vi "PhotonPoseEstimator_Update_All.vi"(9 "Has New Results":bool, 10 "PipelineResult":T1={"Targets"=[], "PhotonMultiTargetPNPResult"={"PhotonPNPResult"={"IsPresent"=FALSE, "bestReprojErr"=0.0, "altReprojErr"=0.0, "ambiguity"=0.0, "Best"={"TRANSLATION3D"={"X"=0.0, "Y"=0.0, "Z"=0.0}, "ROTATION3D"={"Q_quaternion"={"R"=1.0, "V"=[0.0, 0.0, 0.0]}}, "XF"=FALSE}, "Alt"={"TRANSLATION3D"={"X"=0.0, "Y"=0.0, "Z"=0.0}, "ROTATION3D"={"Q_quaternion"={"R"=1.0, "V"=[0.0, 0.0, 0.0]}}, "XF"=FALSE}}, "FiducialIDsUsed"=[]}, "PhotonPipelineMetadata"={"CaptureTimestampMicros"=0, "PublishTimestampMicros"=0, "SequenceID"=0, "TimeSinceLastPong"=0}} {"PhotonMultiTargetPNPResult"."PhotonPNPResult"."Alt"."TRANSLATION3D"."Z" format="%14.3f"; "PhotonMultiTargetPNPResult"."PhotonPNPResult"."Alt"."TRANSLATION3D"."Y" format="%14.3f"; "PhotonMultiTargetPNPResult"."PhotonPNPResult"."Alt"."TRANSLATION3D"."X" format="%14.3f"; "PhotonMultiTargetPNPResult"."PhotonPNPResult"."Best"."TRANSLATION3D"."Z" format="%14.3f"; "PhotonMultiTargetPNPResult"."PhotonPNPResult"."Best"."TRANSLATION3D"."Y" format="%14.3f"; "PhotonMultiTargetPNPResult"."PhotonPNPResult"."Best"."TRANSLATION3D"."X" format="%14.3f"; "Targets"."AltCameraToTarget"."TRANSLATION3D"."Z" format="%14.3f"; "Targets"."AltCameraToTarget"."TRANSLATION3D"."Y" format="%14.3f"; "Targets"."AltCameraToTarget"."TRANSLATION3D"."X" format="%14.3f"; "Targets"."BestCameraToTarget"."TRANSLATION3D"."Z" format="%14.3f"; "Targets"."BestCameraToTarget"."TRANSLATION3D"."Y" format="%14.3f"; "Targets"."BestCameraToTarget"."TRANSLATION3D"."X" format="%14.3f"}, 11 "PhotonPoseEstimator":T14={"LastPose"={"Translation3d"={"X"=0.0, "Y"=0.0, "Z"=0.0}, "Rotation3d"={"Q_quaternion"={"R"=1.0, "V"=[0.0, 0.0, 0.0]}}}, "ReferencePose"={"Translation3d"={"X"=0.0, "Y"=0.0, "Z"=0.0}, "Rotation3d"={"Q_quaternion"={"R"=1.0, "V"=[0.0, 0.0, 0.0]}}}, "FieldTags"={"AprilTagMap"={}, "FieldLength"=0.0, "FieldWidth"=0.0, "OriginPosition "=enum."kBlueAllianceWallRightSide,", "OriginPose3d"={"Translation3d"={"X"=0.0, "Y"=0.0, "Z"=0.0}, "Rotation3d"={"Q_quaternion"={"R"=1.0, "V"=[0.0, 0.0, 0.0]}}}}, "PrimaryStratety"=enum."LOWEST_AMBIGUITY", "Camera"="", "RobotToCamera"={"TRANSLATION3D"={"X"=0.0, "Y"=0.0, "Z"=0.0}, "ROTATION3D"={"Q_quaternion"={"R"=1.0, "V"=[0.0, 0.0, 0.0]}}, "XF"=FALSE}, "ReportedErrors"=[], "HighestAmbiguity"=10.0, "MultiTagFallbackStrategy"=enum."LOWEST_AMBIGUITY", "PoseCacheTimeoutSec"=-1.0, "PhotonTargetModel"={"Vertices"=[], "IsPlaner"=FALSE, "IsSpherical"=FALSE}, "BaseNTName"="/photonvision"} {"PhotonTargetModel"."Vertices"."Z" format="%14.3f"; "PhotonTargetModel"."Vertices"."Y" format="%14.3f"; "PhotonTargetModel"."Vertices"."X" format="%14.3f"; "RobotToCamera"."TRANSLATION3D"."Z" format="%14.3f"; "RobotToCamera"."TRANSLATION3D"."Y" format="%14.3f"; "RobotToCamera"."TRANSLATION3D"."X" format="%14.3f"; "FieldTags"."OriginPose3d"."Translation3d"."Z" format="%14.3f"; "FieldTags"."OriginPose3d"."Translation3d"."Y" format="%14.3f"; "FieldTags"."OriginPose3d"."Translation3d"."X" format="%14.3f"; "ReferencePose"."Translation3d"."Z" format="%14.3f"; "ReferencePose"."Translation3d"."Y" format="%14.3f"; "ReferencePose"."Translation3d"."X" format="%14.3f"; "LastPose"."Translation3d"."Z" format="%14.3f"; "LastPose"."Translation3d"."Y" format="%14.3f"; "LastPose"."Translation3d"."X" format="%14.3f"}) -> (1 "Pos Found":bool, 2 "PhotonEstimatedRobotPose":T11={"EstimatedPose"={"Translation3d"={"X"=0.0, "Y"=0.0, "Z"=0.0}, "Rotation3d"={"Q_quaternion"={"R"=1.0, "V"=[0.0, 0.0, 0.0]}}}, "TimeStamp_Seconds"=0.0, "targetsUsed"=[], "Strategy"=enum."LOWEST_AMBIGUITY"} {"targetsUsed"."AltCameraToTarget"."TRANSLATION3D"."Z" format="%14.3f"; "targetsUsed"."AltCameraToTarget"."TRANSLATION3D"."Y" format="%14.3f"; "targetsUsed"."AltCameraToTarget"."TRANSLATION3D"."X" format="%14.3f"; "targetsUsed"."BestCameraToTarget"."TRANSLATION3D"."Z" format="%14.3f"; "targetsUsed"."BestCameraToTarget"."TRANSLATION3D"."Y" format="%14.3f"; "targetsUsed"."BestCameraToTarget"."TRANSLATION3D"."X" format="%14.3f"; "EstimatedPose"."Translation3d"."Z" format="%14.3f"; "EstimatedPose"."Translation3d"."Y" format="%14.3f"; "EstimatedPose"."Translation3d"."X" format="%14.3f"}, 3 "out PhotonPoseEstimator":T14={"LastPose"={"Translation3d"={"X"=0.0, "Y"=0.0, "Z"=0.0}, "Rotation3d"={"Q_quaternion"={"R"=1.0, "V"=[0.0, 0.0, 0.0]}}}, "ReferencePose"={"Translation3d"={"X"=0.0, "Y"=0.0, "Z"=0.0}, "Rotation3d"={"Q_quaternion"={"R"=1.0, "V"=[0.0, 0.0, 0.0]}}}, "FieldTags"={"AprilTagMap"={}, "FieldLength"=0.0, "FieldWidth"=0.0, "OriginPosition "=enum."kBlueAllianceWallRightSide,", "OriginPose3d"={"Translation3d"={"X"=0.0, "Y"=0.0, "Z"=0.0}, "Rotation3d"={"Q_quaternion"={"R"=1.0, "V"=[0.0, 0.0, 0.0]}}}}, "PrimaryStratety"=enum."LOWEST_AMBIGUITY", "Camera"="", "RobotToCamera"={"TRANSLATION3D"={"X"=0.0, "Y"=0.0, "Z"=0.0}, "ROTATION3D"={"Q_quaternion"={"R"=1.0, "V"=[0.0, 0.0, 0.0]}}, "XF"=FALSE}, "ReportedErrors"=[], "HighestAmbiguity"=10.0, "MultiTagFallbackStrategy"=enum."LOWEST_AMBIGUITY", "PoseCacheTimeoutSec"=-1.0, "PhotonTargetModel"={"Vertices"=[], "IsPlaner"=FALSE, "IsSpherical"=FALSE}, "BaseNTName"="/photonvision"} {"PhotonTargetModel"."Vertices"."Z" format="%14.3f"; "PhotonTargetModel"."Vertices"."Y" format="%14.3f"; "PhotonTargetModel"."Vertices"."X" format="%14.3f"; "RobotToCamera"."TRANSLATION3D"."Z" format="%14.3f"; "RobotToCamera"."TRANSLATION3D"."Y" format="%14.3f"; "RobotToCamera"."TRANSLATION3D"."X" format="%14.3f"; "FieldTags"."OriginPose3d"."Translation3d"."Z" format="%14.3f"; "FieldTags"."OriginPose3d"."Translation3d"."Y" format="%14.3f"; "FieldTags"."OriginPose3d"."Translation3d"."X" format="%14.3f"; "ReferencePose"."Translation3d"."Z" format="%14.3f"; "ReferencePose"."Translation3d"."Y" format="%14.3f"; "ReferencePose"."Translation3d"."X" format="%14.3f"; "LastPose"."Translation3d"."Z" format="%14.3f"; "LastPose"."Translation3d"."Y" format="%14.3f"; "LastPose"."Translation3d"."X" format="%14.3f"})   [LabVIEW 2019, in "PhotonVisionLib.lvlib"]
doc: "Provided data from polling a camera, updates the estimated position of the robot. Returns empty if:\n - New data has not been received since the last call to update.\n - No targets were found from the camera\n - There is no camera set\n\n** DEPRECATED 2026 ** Functions that use the strategy enum are being deprecated. Use the individual strategy EXECUTE or ESTIMATE functions instead.\n\nInputs:\n -- PhotonPoseEstimator -- data cluster -- Data guiding how the position determination is done.\n -- PipelineResults -- data cluster -- Data provided from PhotonCamera_GetLatestResults.\n -- HasResults -- boolean - TRUE if targets have been identified in the Pipeline results. This can be provided by PhotonCamera_GetLatestResults.\n -- cameraMatrix -- matrix -- Camera calibration data that can be used in the case of no assigned PhotonCamera.\n -- distCoeffs -- matrix -- Camera calibration data that can be used in the case of no assigned PhotonCamera\n\nOutputs:\n -- PhotonPoseEstimator -- data cluster -- Updated data cluster.\n -- PhotonEstimatedRobotPose -- data cluster -- Estimated robot position, timestamp, and targets used to create the estimte.\n -- PosFound -- boolean -- A position has been determined."
uses:
  PhotonVisionLib.lvlib
  TypeDef/PhotonPoseEstimatorType.ctl
  <vilib>/Rock Robotics/WPI/ThirdParty/JAS_Junk/TrajLib/TypeDef/POSE3D.ctl
  <vilib>/Rock Robotics/WPI/ThirdParty/JAS_Junk/TrajLib/TypeDef/TRANSLATION3D.ctl
  <vilib>/Rock Robotics/WPI/ThirdParty/JAS_Junk/TrajLib/TypeDef/ROTATION3D.ctl
  <vilib>/Rock Robotics/WPI/ThirdParty/JAS_Junk/TrajLib/TypeDef/QUATERNION.ctl
  <vilib>/Rock Robotics/WPI/ThirdParty/JAS_Junk/TrajLib/TypeDef/AprilTagFieldLayout.ctl
  <vilib>/Rock Robotics/WPI/ThirdParty/JAS_Junk/TrajLib/TypeDef/AprilTag.ctl
  <vilib>/Rock Robotics/WPI/ThirdParty/JAS_Junk/TrajLib/Enum/AprilTagFieldLayoutOrignPosition_ENUM.ctl
  Enum/PhotonPoseStrategy_ENUM.ctl
  <vilib>/Rock Robotics/WPI/ThirdParty/JAS_Junk/TrajLib/TypeDef/TRANSFORM3D.ctl
  TypeDef/PhotonTargetModel.ctl
  TypeDef/PhotonEstimatedRobotPoseType.ctl
  TypeDef/PhotonTrackedTargetType.ctl
  TypeDef/TargetCornerType.ctl
  TypeDef/PhotonPipelineResultType.ctl
  TypeDef/PhotonMultiTargetPNPResultType.ctl
  TypeDef/PhotonPNPResultType.ctl
  TypeDef/PhotonPipelineMetadataType.ctl
  <vilib>/Rock Robotics/WPI/ThirdParty/JAS_Junk/TrajLib/VI/Rotation3d_Create_AxisAngle.vi
  <vilib>/Rock Robotics/WPI/ThirdParty/JAS_Junk/TrajLib/VI/Pose3d_New.vi
  PhotonPipelineResult_HasTargets.vi
  PhotonPipelineResult_GetTargets.vi
  PhotonTrackedTarget_GetPoseAmbiguity.vi
  PhotonTrackedTarget_GetFiducialId.vi
  PhotonPoseEstimator_GetFieldTags.vi
  <vilib>/Rock Robotics/WPI/ThirdParty/JAS_Junk/TrajLib/VI/AprilTagFieldLayout_GetTagPose.vi
  <vilib>/Rock Robotics/WPI/ThirdParty/JAS_Junk/TrajLib/VI/Pose3d_TransformBy.vi
  PhotonTrackedTarget_GetBestCameraToTarget.vi
  <vilib>/Rock Robotics/WPI/ThirdParty/JAS_Junk/TrajLib/VI/Transform3d_Inverse.vi
  PhotonPoseEstimator_GetRobotToCameraTransform.vi
  PhotonPoseEstimator_GetHighestAmbiguity.vi
  PhotonEstimatedRobotPose_New.vi
  PhotonPoseEstimator_Strategy_closestToCameraHeight_calc.vi
  PhotonTrackedTarget_GetAltCameraToTarget.vi
  PhotonPoseEstimator_Strategy_closestToReferencePose_calc.vi
  PhotonPoseEstimator_Strategy_averageBestTargets_calc.vi
  <vilib>/Rock Robotics/WPI/ThirdParty/JAS_Junk/TrajLib/VI/Rotation3d_Plus.vi
  <vilib>/Rock Robotics/WPI/ThirdParty/JAS_Junk/TrajLib/VI/Translation3d_Plus.vi
  <vilib>/Rock Robotics/WPI/ThirdParty/JAS_Junk/TrajLib/VI/Translation3d_Times.vi
  <vilib>/Rock Robotics/WPI/ThirdParty/JAS_Junk/TrajLib/VI/Rotation3d_Times.vi
  <vilib>/Rock Robotics/WPI/ThirdParty/JAS_Junk/TrajLib/VI/Rotation3d_Create_Default.vi
  <vilib>/Rock Robotics/WPI/ThirdParty/JAS_Junk/TrajLib/VI/Translation3d_Create_Default.vi
  <vilib>/Rock Robotics/WPI/ThirdParty/JAS_Junk/TrajLib/VI/Pose3d_New_Trans3dRot3d.vi
  <vilib>/Rock Robotics/WPI/ThirdParty/JAS_Junk/TrajLib/VI/Pose3d_New_Default.vi
  <vilib>/Rock Robotics/WPI/ThirdParty/JAS_Junk/TrajLib/VI/Pose3d_Plus.vi
  <vilib>/Rock Robotics/WPI/ThirdParty/JAS_Junk/TrajLib/VI/Pose3d_RelativeTo.vi
  <vilib>/Rock Robotics/WPI/ThirdParty/JAS_Junk/TrajLib/VI/AprilTagFieldLayout_GetOriginPosition.vi
  PhotonPipelineResult_GetMultiTagResult.vi
  PhotonPipelineResult_GetBestTarget.vi
  PhotonTrackedTarget_GetPitch.vi
  PhotonTrackedTarget_GetYaw.vi
  <vilib>/Rock Robotics/WPI/ThirdParty/JAS_Junk/TrajLib/VI/Rotation3d_Create_RollPitchYaw.vi
  <vilib>/Rock Robotics/WPI/ThirdParty/JAS_Junk/TrajLib/Units_DegreesToRadians.vi
  <vilib>/Rock Robotics/WPI/ThirdParty/JAS_Junk/TrajLib/VI/Transform3d_GetTranslation3d.vi
  <vilib>/Rock Robotics/WPI/ThirdParty/JAS_Junk/TrajLib/VI/Translation3d_GetNorm.vi
  <vilib>/Rock Robotics/WPI/ThirdParty/JAS_Junk/TrajLib/VI/Translation3d_Create_DistAng.vi
  <vilib>/Rock Robotics/WPI/ThirdParty/JAS_Junk/TrajLib/VI/Translation3d_RotateBy.vi
  <vilib>/Rock Robotics/WPI/ThirdParty/JAS_Junk/TrajLib/VI/Translation3d_ToTranslation2d.vi
  <vilib>/Rock Robotics/WPI/ThirdParty/JAS_Junk/TrajLib/Translation2d_RotateBy.vi
  <vilib>/Rock Robotics/WPI/ThirdParty/JAS_Junk/TrajLib/VI/Transform3d_GetRotation3d.vi
  <vilib>/Rock Robotics/WPI/ThirdParty/JAS_Junk/TrajLib/VI/Pose3d_ToPose2d.vi
  <vilib>/Rock Robotics/WPI/ThirdParty/JAS_Junk/TrajLib/Pose2d_getTranslation.vi
  <vilib>/Rock Robotics/WPI/ThirdParty/JAS_Junk/TrajLib/Translation2d_Plus.vi
  <vilib>/Rock Robotics/WPI/ThirdParty/JAS_Junk/TrajLib/Translation2d_UnaryMinus.vi
  <vilib>/Rock Robotics/WPI/ThirdParty/JAS_Junk/TrajLib/Pose2d_New_TRRO.vi
  <vilib>/Rock Robotics/WPI/ThirdParty/JAS_Junk/TrajLib/VI/Pose3d_New_Pose2d.vi
  <vilib>/Rock Robotics/WPI/ThirdParty/JAS_Junk/TrajLib/VI/TimeInterpRotation2d_GetSample.vi
  PhotonPoseEstimator_GetHeadingBuffer.vi
  <vilib>/Rock Robotics/WPI/ThirdParty/JAS_Junk/TrajLib/VI/Quaternion_New.vi
  <vilib>/Rock Robotics/WPI/ThirdParty/JAS_Junk/TrajLib/VI/Vector_Norm.vi
  <vilib>/Rock Robotics/WPI/ThirdParty/JAS_Junk/TrajLib/VecBuilder_ArrayBy1Fill.vi
  <vilib>/Rock Robotics/WPI/ThirdParty/JAS_Junk/TrajLib/VI/Translation3d_Create.vi
  PhotonPipelineResult_GetTargetCount.vi
  <vilib>/Rock Robotics/WPI/ThirdParty/JAS_Junk/TrajLib/VI/AprilTag_GetAll.vi
  <vilib>/Rock Robotics/WPI/ThirdParty/JAS_Junk/TrajLib/VI/Pose3d_getTranslation3d.vi
  <vilib>/Rock Robotics/WPI/ThirdParty/JAS_Junk/TrajLib/VI/Pose3d_getRotation3d.vi
  <vilib>/Rock Robotics/WPI/ThirdParty/JAS_Junk/TrajLib/VI/Rotation3d_ToRotation2d.vi
  <vilib>/Rock Robotics/WPI/ThirdParty/JAS_Junk/TrajLib/Transform2d_Create_TransRot.vi
  <vilib>/Rock Robotics/WPI/ThirdParty/JAS_Junk/TrajLib/VI/Transform3d_Create_Trans3dRot3d.vi
  <vilib>/Rock Robotics/WPI/ThirdParty/JAS_Junk/TrajLib/VI/Rotation3d_UnaryMinus.vi
  <vilib>/Rock Robotics/WPI/ThirdParty/JAS_Junk/TrajLib/VI/Translation3d_UnaryMinus.vi
  <vilib>/Rock Robotics/WPI/ThirdParty/JAS_Junk/TrajLib/VI/Transform3d_GetXYZ.vi
  <vilib>/Rock Robotics/WPI/ThirdParty/JAS_Junk/TrajLib/VI/Pose3d_getXYZ.vi
  PhotonPoseEstimator_CalcDifference.vi
  <vilib>/Rock Robotics/WPI/ThirdParty/JAS_Junk/TrajLib/VI/Rotation3d_RotateBy.vi
  <vilib>/Rock Robotics/WPI/ThirdParty/JAS_Junk/TrajLib/VI/Translation3d_GetXYZ.vi
  <vilib>/Rock Robotics/WPI/ThirdParty/JAS_Junk/TrajLib/VI/Rotation3d_GetQuaterion.vi
  <vilib>/Rock Robotics/WPI/ThirdParty/JAS_Junk/TrajLib/VI/Quaternion_Get_Vect.vi
  <vilib>/Rock Robotics/WPI/ThirdParty/JAS_Junk/TrajLib/VI/Quaternion_Get_W.vi
  <vilib>/Rock Robotics/WPI/ThirdParty/JAS_Junk/TrajLib/VI/Quaternion_New_Default.vi
  <vilib>/Rock Robotics/WPI/ThirdParty/JAS_Junk/TrajLib/VI/Transform3d_Create_Pose3dPose3d.vi
  <vilib>/Rock Robotics/WPI/ThirdParty/JAS_Junk/TrajLib/Conv_Deg_Radians.vi
  <vilib>/Rock Robotics/WPI/ThirdParty/JAS_Junk/TrajLib/VI/Quaternion_Times.vi
  <vilib>/Rock Robotics/WPI/ThirdParty/JAS_Junk/TrajLib/VI/Quaternion_Inverse.vi
  <vilib>/Rock Robotics/WPI/ThirdParty/JAS_Junk/TrajLib/VI/Quaternion_Get_All.vi
  <vilib>/Rock Robotics/WPI/ThirdParty/JAS_Junk/TrajLib/Translation2d_Create.vi
  <vilib>/Rock Robotics/WPI/ThirdParty/JAS_Junk/TrajLib/Pose2d_getXYAngle.vi
  <vilib>/Rock Robotics/WPI/ThirdParty/JAS_Junk/TrajLib/Rotation2d_Interpolate.vi
  <vilib>/Rock Robotics/WPI/ThirdParty/JAS_Junk/TrajLib/MatBuilder_Create.vi
  <vilib>/Rock Robotics/WPI/ThirdParty/JAS_Junk/TrajLib/Rotation2d_CreateAngle.vi
  <vilib>/Rock Robotics/WPI/ThirdParty/JAS_Junk/TrajLib/VI/Rotation3d_GetXYZ.vi
  <vilib>/Rock Robotics/WPI/ThirdParty/JAS_Junk/TrajLib/VI/Rotation3d_Create_Quaternion.vi
  <vilib>/Rock Robotics/WPI/ThirdParty/JAS_Junk/TrajLib/VI/Translation3d_GetDistance.vi
  <vilib>/Rock Robotics/WPI/ThirdParty/JAS_Junk/TrajLib/VI/Translation3d_Minus.vi
  <vilib>/Rock Robotics/WPI/ThirdParty/JAS_Junk/TrajLib/VI/Rotation3d_Minus.vi
  <vilib>/Rock Robotics/WPI/ThirdParty/JAS_Junk/TrajLib/Rotation2d_Plus.vi
  <vilib>/Rock Robotics/WPI/ThirdParty/JAS_Junk/TrajLib/Rotation2d_Minus.vi
  <vilib>/Rock Robotics/WPI/ThirdParty/JAS_Junk/TrajLib/MathUtil_Clamp.vi
  <vilib>/Rock Robotics/WPI/ThirdParty/JAS_Junk/TrajLib/Rotation2d_Times.vi
  <vilib>/Rock Robotics/WPI/ThirdParty/JAS_Junk/TrajLib/VI/Quaternion_Normalize.vi
  <vilib>/Rock Robotics/WPI/ThirdParty/JAS_Junk/TrajLib/Rotation2d_RotateBy.vi
  <vilib>/Rock Robotics/WPI/ThirdParty/JAS_Junk/TrajLib/Rotation2d_UnaryMinus.vi
  <vilib>/Rock Robotics/WPI/ThirdParty/JAS_Junk/TrajLib/Rotation2d_CreateXY.vi
  <vilib>/Rock Robotics/WPI/ThirdParty/JAS_Junk/TrajLib/Util_CalcDist.vi
  PhotonVision_Globals.vi
  <vilib>/gmath/interp.llb/Search Ordered Table.vi
  <vilib>/Rock Robotics/WPI/ThirdParty/JAS_Junk/TrajLib/Trajectory_Library.lvlib
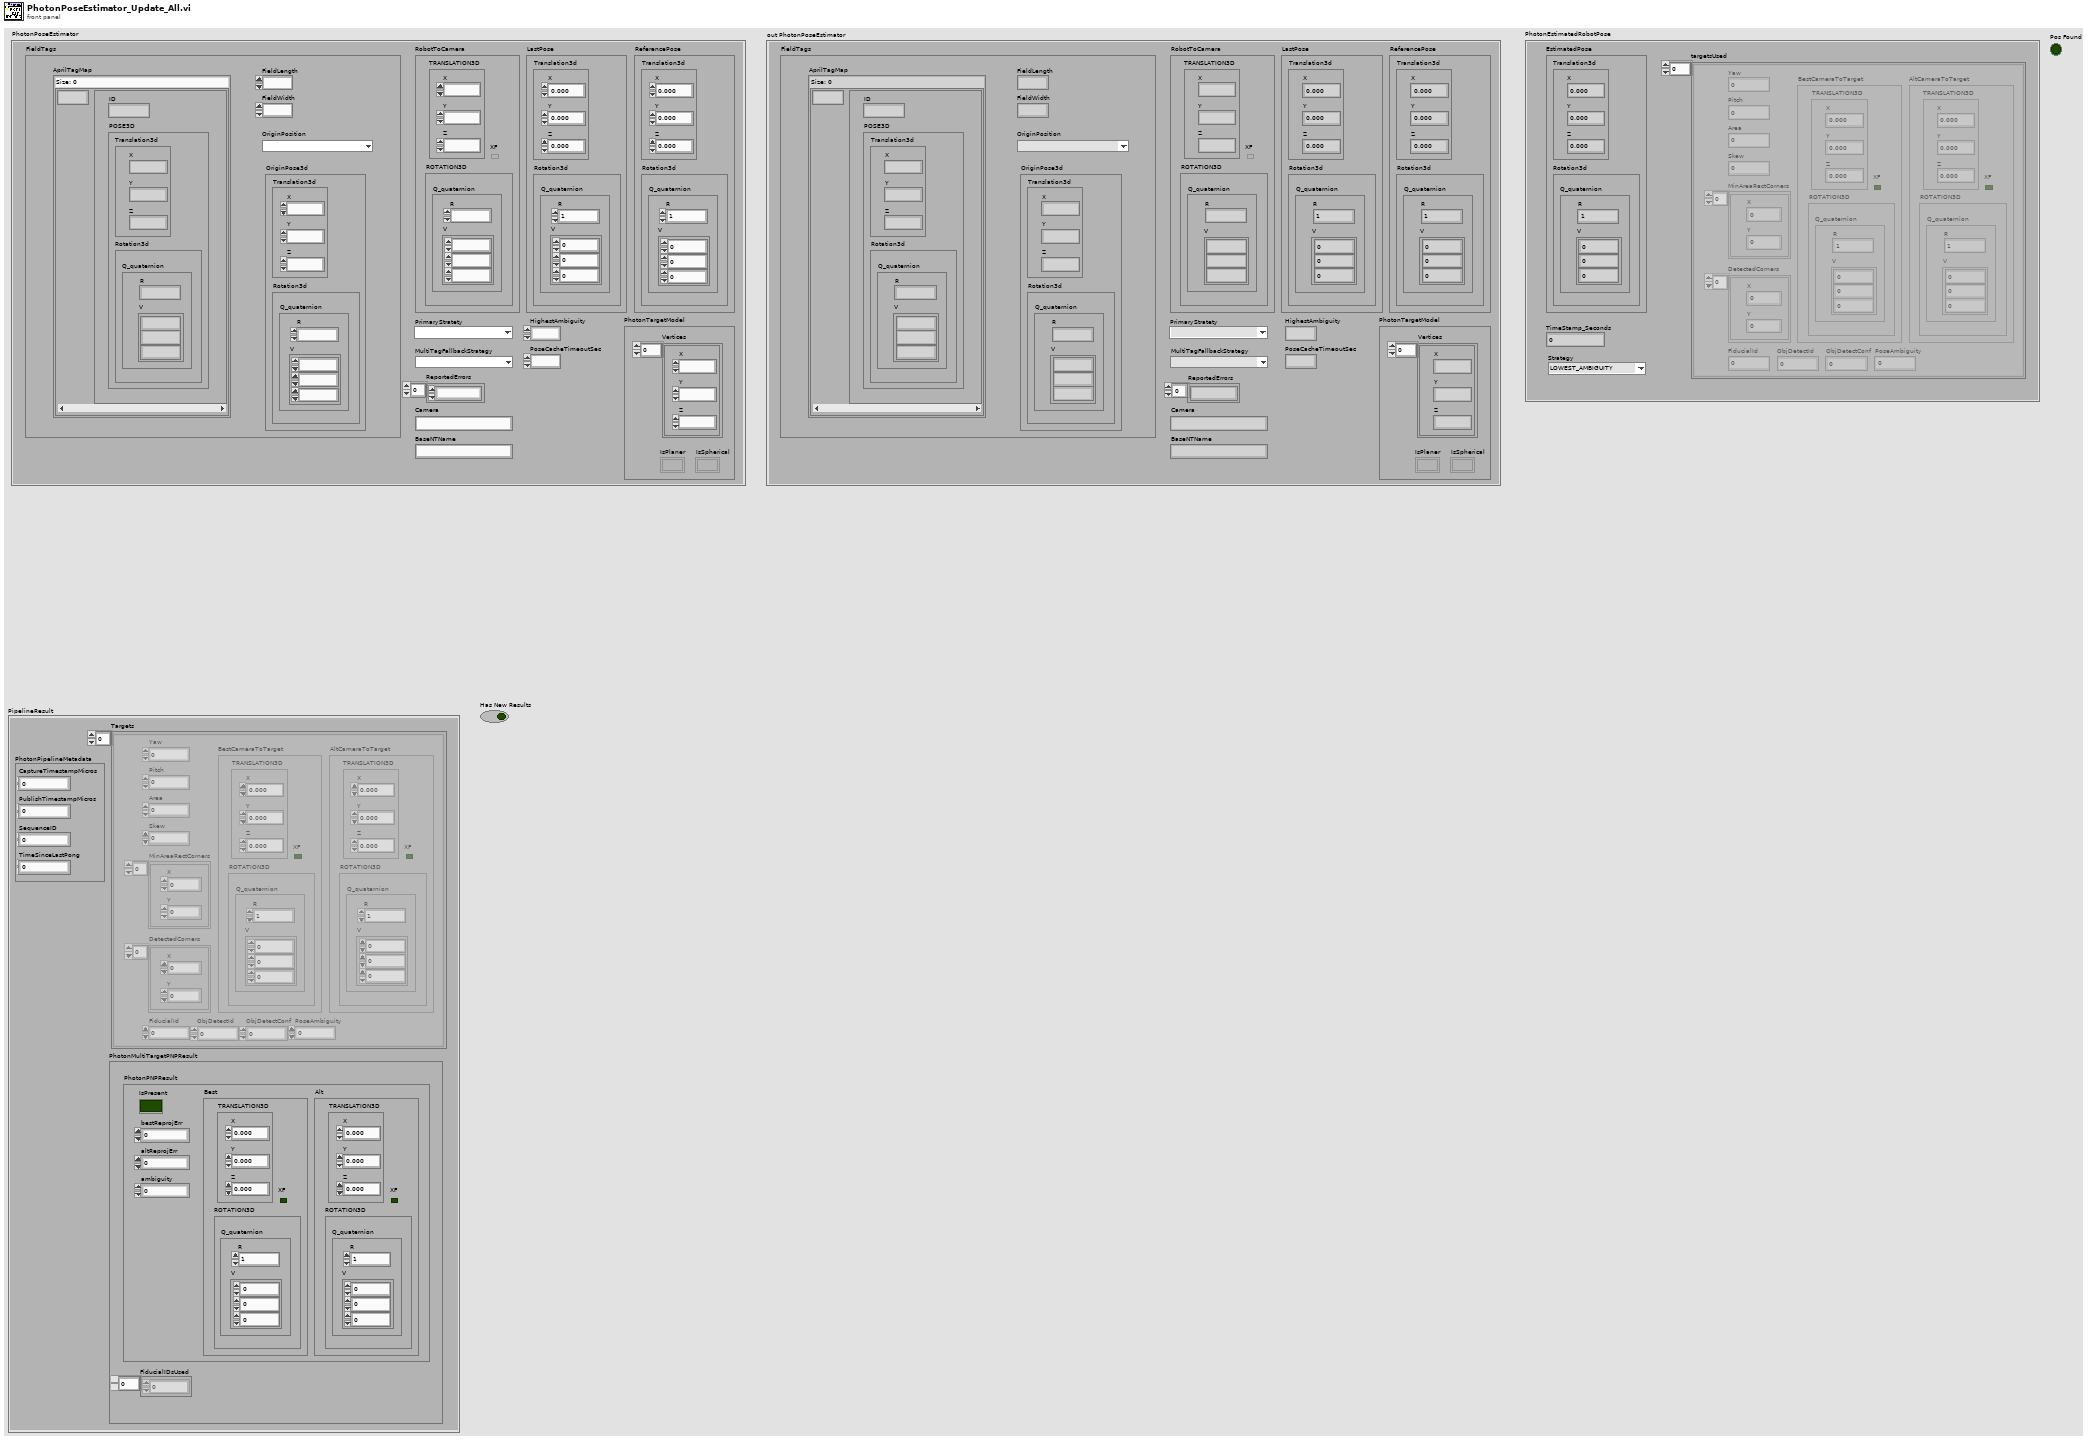
[diagram p1: front panel]
types:
  T1 = typedef "PhotonVisionLib.lvlib/PhotonPipelineResultType.ctl" = cluster{"Targets":T2[], "PhotonMultiTargetPNPResult":T8, "PhotonPipelineMetadata":T10}
  T2 = typedef "PhotonVisionLib.lvlib/PhotonTrackedTargetType.ctl" = cluster{"Yaw":dbl, "Pitch":dbl, "Area":dbl, "Skew":dbl, "MinAreaRectCorners":T3[], "BestCameraToTarget":T4, "FiducialId":i32, "AltCameraToTarget":T4, "PoseAmbiguity":dbl, "DetectedCorners":T3[], "ObjDetectId":i32, "ObjDetectConf":sgl}
  T3 = typedef "PhotonVisionLib.lvlib/TargetCornerType.ctl" = cluster{"X":dbl, "Y":dbl}
  T4 = typedef "Trajectory_Library.lvlib/TRANSFORM3D.ctl" = cluster{"TRANSLATION3D":T5, "ROTATION3D":T6, "XF":bool}
  T5 = typedef "Trajectory_Library.lvlib/TRANSLATION3D.ctl" = cluster{"X":dbl, "Y":dbl, "Z":dbl}
  T6 = typedef "Trajectory_Library.lvlib/ROTATION3D.ctl" = cluster{"Q_quaternion":T7}
  T7 = typedef "Trajectory_Library.lvlib/QUATERNION.ctl" = cluster{"R":dbl, "V":dbl[]}
  T8 = typedef "PhotonVisionLib.lvlib/PhotonMultiTargetPNPResultType.ctl" = cluster{"PhotonPNPResult":T9, "FiducialIDsUsed":i16[]}
  T9 = typedef "PhotonVisionLib.lvlib/PhotonPNPResultType.ctl" = cluster{"IsPresent":bool, "bestReprojErr":dbl, "altReprojErr":dbl, "ambiguity":dbl, "Best":T4, "Alt":T4}
  T10 = typedef "PhotonVisionLib.lvlib/PhotonPipelineMetadataType.ctl" = cluster{"CaptureTimestampMicros":i64, "PublishTimestampMicros":i64, "SequenceID":i64, "TimeSinceLastPong":i64}
  T11 = typedef "PhotonVisionLib.lvlib/PhotonEstimatedRobotPoseType.ctl" = cluster{"EstimatedPose":T12, "TimeStamp_Seconds":dbl, "targetsUsed":T2[], "Strategy":T13}
  T12 = typedef "Trajectory_Library.lvlib/POSE3D.ctl" = cluster{"Translation3d":T5, "Rotation3d":T6}
  T13 = typedef "PhotonVisionLib.lvlib/PhotonPoseStrategy_ENUM.ctl" = enum16{"LOWEST_AMBIGUITY", "CLOSEST_TO_CAMERA_HEIGHT", "CLOSEST_TO_REFERENCE_POSE", "CLOSEST_TO_LAST_POSE", "AVERAGE_BEST_TARGETS", "MULTI_TAG_PNP_ON_COPROCESSOR", "MULTI_TAG_PNP_ON_RIO", "PNP_DISTANCE_TRIG_SOLVE", "CONSTRAINED_SOLVEPNP"}
  T14 = typedef "PhotonVisionLib.lvlib/PhotonPoseEstimatorType.ctl" = cluster{"LastPose":T12, "ReferencePose":T12, "FieldTags":T15, "PrimaryStratety":T13, "Camera":string, "RobotToCamera":T4, "ReportedErrors":dbl[], "HighestAmbiguity":dbl, "MultiTagFallbackStrategy":T13, "PoseCacheTimeoutSec":dbl, "PhotonTargetModel":T18, "BaseNTName":string}
  T15 = typedef "Trajectory_Library.lvlib/AprilTagFieldLayout.ctl" = cluster{"AprilTagMap":map{i32, T16}, "FieldLength":dbl, "FieldWidth":dbl, "OriginPosition ":T17, "OriginPose3d":T12}
  T16 = typedef "Trajectory_Library.lvlib/AprilTag.ctl" = cluster{"ID":i32, "POSE3D":T12}
  T17 = typedef "Trajectory_Library.lvlib/AprilTagFieldLayoutOrignPosition_ENUM.ctl" = enum16{"kBlueAllianceWallRightSide,", "kRedAllianceWallRightSide,"}
  T18 = typedef "PhotonVisionLib.lvlib/PhotonTargetModel.ctl" = cluster{"Vertices":T5[], "IsPlaner":bool, "IsSpherical":bool}
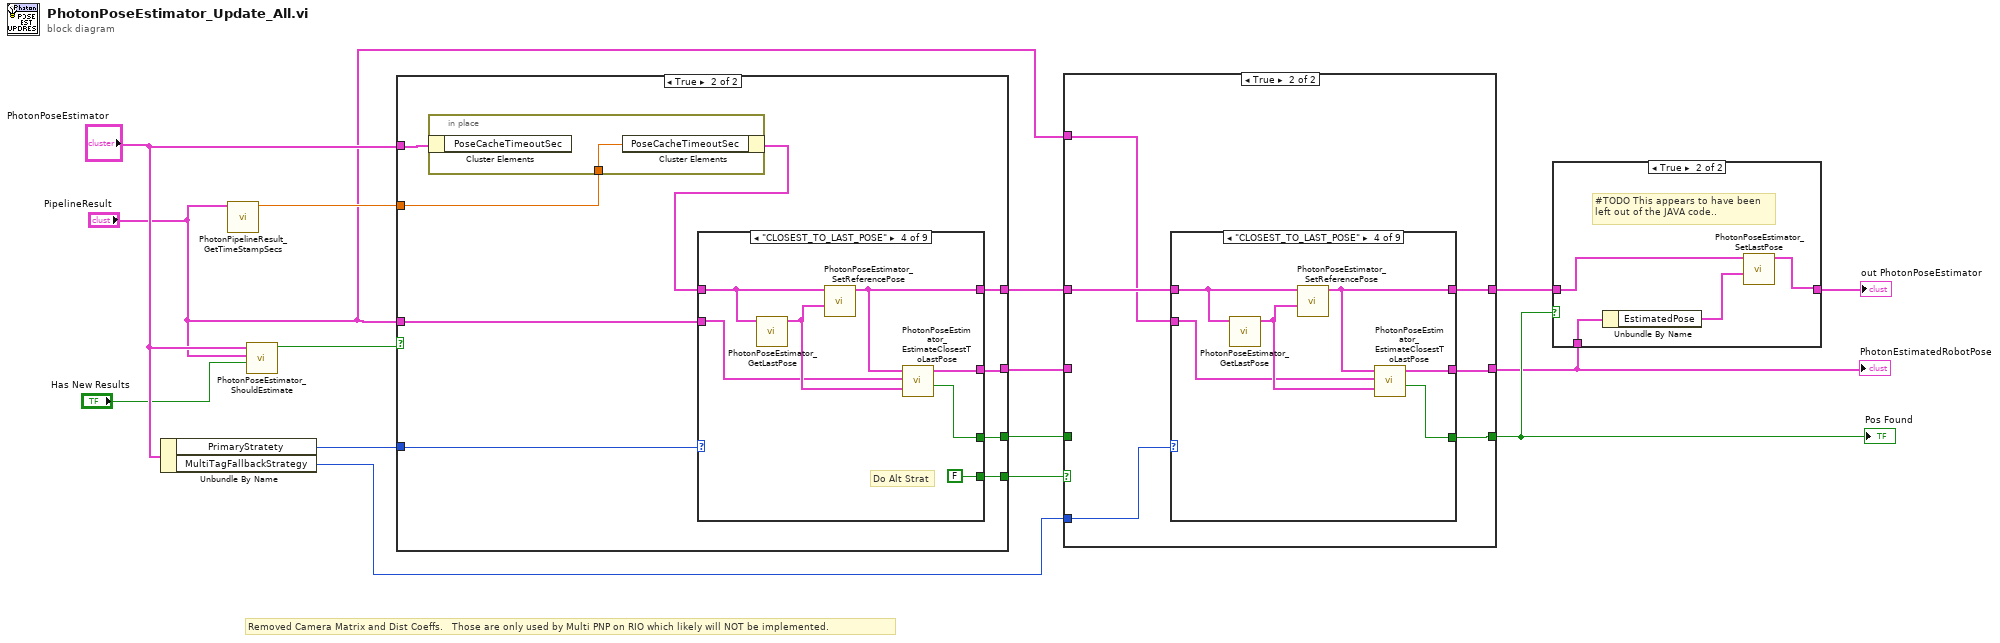
[diagram p0: block diagram]
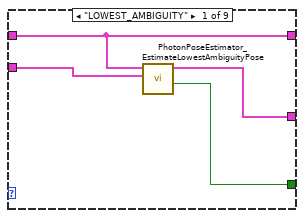
[diagram p3: hidden frame]
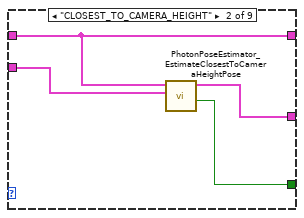
[diagram p4: hidden frame]
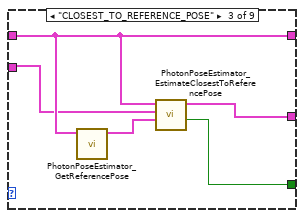
[diagram p5: hidden frame]
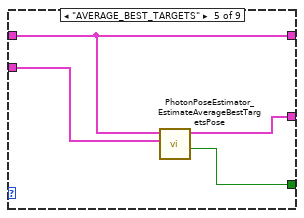
[diagram p6: hidden frame]
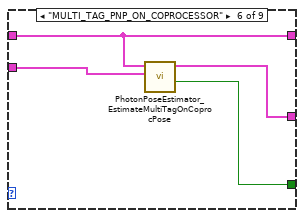
[diagram p7: hidden frame]
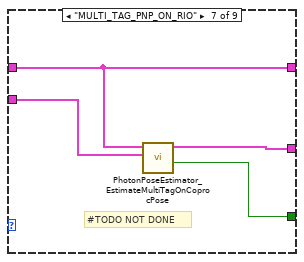
[diagram p8: hidden frame]
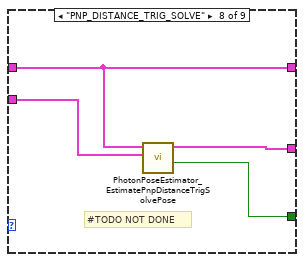
[diagram p9: hidden frame]
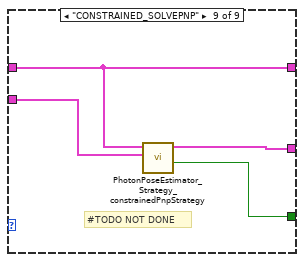
[diagram p10: hidden frame]
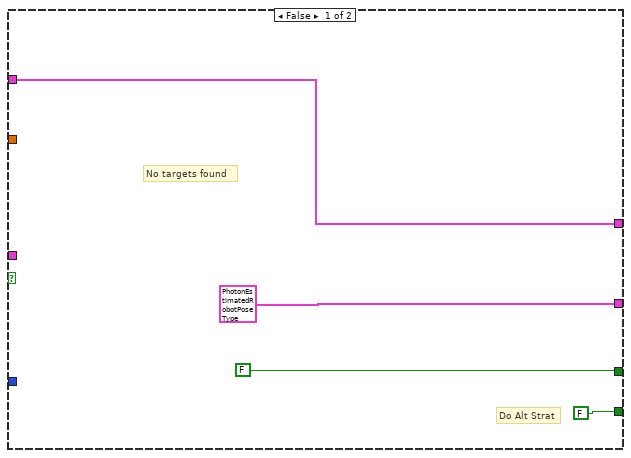
[diagram p11: hidden frame]
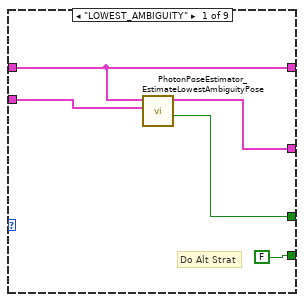
[diagram p12: hidden frame]
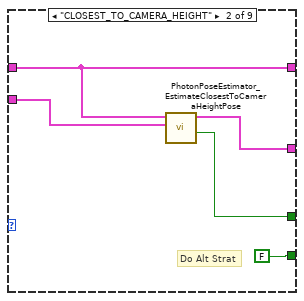
[diagram p13: hidden frame]
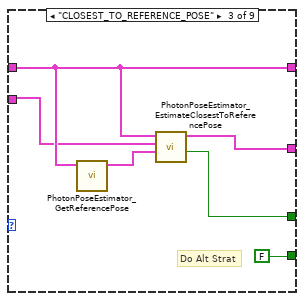
[diagram p14: hidden frame]
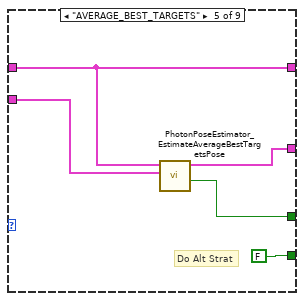
[diagram p15: hidden frame]
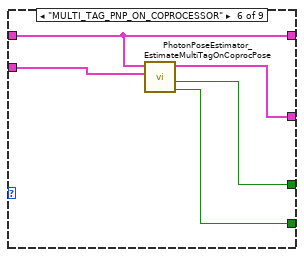
[diagram p16: hidden frame]
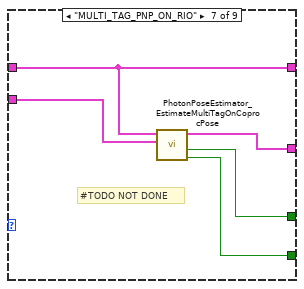
[diagram p17: hidden frame]
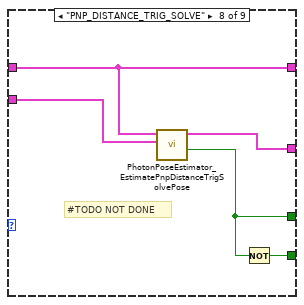
[diagram p18: hidden frame]
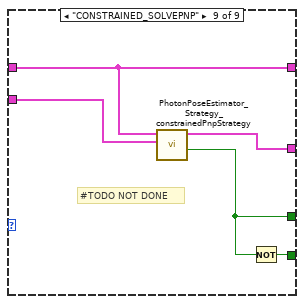
[diagram p19: hidden frame]
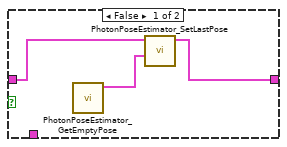
[diagram p20: hidden frame]
diagram:
  # "Removed Camera Matrix and Dist Coeffs.   Those are only used by Multi PNP on RIO which likely will NOT be implemented."
  n1 = Unbundle By Name("PhotonPoseEstimator") -> ("PrimaryStratety"=w15:T13, "MultiTagFallbackStrategy"=w6:T13)
  n2 = call "PhotonPipelineResult_GetTimeStampSecs.vi"("PhotonPipelineResult"="PipelineResult") -> ("TimeStampSec"=w5:dbl)  [unwired: 10 in]
  n3 = call "PhotonPoseEstimator_ShouldEstimate.vi"("HasResults"="Has New Results", "PipelineResult"="PipelineResult", "PhotonPoseEstimator"="PhotonPoseEstimator") -> ("ShouldEstimate"=w1:bool)  [unwired: 8 in]
  n4 = case shown="True" w1 {
    tunnel: [w19 w26] -> w8
    tunnel: "PhotonPoseEstimator" -> [w19 w23]
    tunnel: [T11 {"EstimatedPose"={"Translation3d"={"X"=0.0, "Y"=0.0, "Z"=0.0}, "Rotation3d"={"Q_quaternion"={"R"=1.0, "V"=[0.0, 0.0, 0.0]}}}, "TimeStamp_Seconds"=0.0, "targetsUsed"=[], "Strategy"=enum."LOWEST_AMBIGUITY"} ("PhotonEstimatedRobotPose") w24] -> w10
    tunnel: [FALSE w25] -> w12
    tunnel: w15 -> [_ w28]
    tunnel: "PipelineResult" -> [_ w27]
    tunnel: w5 -> [_ w21]
    tunnel: [FALSE ("Do Alt Strategy") w20] -> w13
    frame False {
      # "Do Alt Strat"
      # "No targets found"
    }
    frame True {
      n5 = in-place {
        in-place-border: w21 -> [w29]
        n6 = in-place-cluster #1(w23) -> ()  [unwired: 1 out]
        n7 = in-place-cluster #1("PoseCacheTimeoutSec"=w29) -> (w22:T14)
      }
      n8 = case shown="\"CLOSEST_TO_LAST_POSE\"" w28 {
        tunnel: w27 -> [w31 w36 w41 w48 w54 w61 w66 w71 w76]
        tunnel: w22 -> [w32 w37 w42 w52 w55 w62 w67 w72 w77]
        tunnel: [w32 w37 w42 w47 w55 w62 w67 w72 w77] -> w26
        tunnel: [w34 w38 w43 w49 w56 w59 w64 w68 w73] -> w25
        tunnel: [w33 w39 w44 w50 w57 w60 w65 w70 w75] -> w24
        tunnel: [FALSE ("Do Alt Strategy") FALSE ("Do Alt Strategy") FALSE ("Do Alt Strategy") FALSE ("Do Alt Strategy") FALSE ("Do Alt Strategy") w58 w63 w69 w74] -> w20
        frame "LOWEST_AMBIGUITY" {
          # "Do Alt Strat"
          n9 = call "PhotonPoseEstimator_EstimateLowestAmbiguityPose.vi"("CameraResult"=w31, "PhotoPoseEstimator"=w32) -> ("Pos Found"=w34:bool, "PhotonEstimatedRobotPose"=w33:T11)  [unwired: 8 in]
        }
        frame "CLOSEST_TO_CAMERA_HEIGHT" {
          # "Do Alt Strat"
          n10 = call "PhotonPoseEstimator_EstimateClosestToCameraHeightPose.vi"("CameraResult"=w36, "PhotoPoseEstimator"=w37) -> ("Pos Found"=w38:bool, "PhotonEstimatedRobotPose"=w39:T11)  [unwired: 8 in]
        }
        frame "CLOSEST_TO_REFERENCE_POSE" {
          # "Do Alt Strat"
          n11 = call "PhotonPoseEstimator_GetReferencePose.vi"("PhotonPoseEstimator"=w42) -> ("ReferencePose"=w45:T12)  [unwired: 10 in]
          n12 = call "PhotonPoseEstimator_EstimateClosestToReferencePose.vi"("ReferencePose"=w45, "CameraResult"=w41, "PhotoPoseEstimator"=w42) -> ("Pos Found"=w43:bool, "PhotonEstimatedRobotPose"=w44:T11)  [unwired: 7 in]
        }
        frame "CLOSEST_TO_LAST_POSE" {
          # "Do Alt Strat"
          n13 = call "PhotonPoseEstimator_GetLastPose.vi"("PhotonPoseEstimator"=w52) -> ("LastPose"=w51:T12)  [unwired: 10 in]
          n14 = call "PhotonPoseEstimator_SetReferencePose.vi"("ReferencePose"=w51, "PhotonPoseEstimator"=w52) -> ("out PhotonPoseEstimator"=w47:T14)  [unwired: 9 in]
          n15 = call "PhotonPoseEstimator_EstimateClosestToLastPose.vi"("LastPose"=w51, "CameraResult"=w48, "PhotoPoseEstimator"=w47) -> ("Pos Found"=w49:bool, "PhotonEstimatedRobotPose"=w50:T11)  [unwired: 7 in]
        }
        frame "AVERAGE_BEST_TARGETS" {
          # "Do Alt Strat"
          n16 = call "PhotonPoseEstimator_EstimateAverageBestTargetsPose.vi"("CameraResult"=w54, "PhotoPoseEstimator"=w55) -> ("Pos Found"=w56:bool, "PhotonEstimatedRobotPose"=w57:T11)  [unwired: 8 in]
        }
        frame "MULTI_TAG_PNP_ON_COPROCESSOR" {
          n17 = call "PhotonPoseEstimator_EstimateMultiTagOnCoprocPose.vi"("CameraResult"=w61, "PhotoPoseEstimator"=w62) -> ("Do Alt Strategy"=w58:bool, "Pos Found"=w59:bool, "PhotonEstimatedRobotPose"=w60:T11)  [unwired: 7 in]
        }
        frame "MULTI_TAG_PNP_ON_RIO" {
          # "#TODO NOT DONE"
          n18 = call "PhotonPoseEstimator_EstimateMultiTagOnCoprocPose.vi"("CameraResult"=w66, "PhotoPoseEstimator"=w67) -> ("Do Alt Strategy"=w63:bool, "Pos Found"=w64:bool, "PhotonEstimatedRobotPose"=w65:T11)  [unwired: 7 in]
        }
        frame "PNP_DISTANCE_TRIG_SOLVE" {
          # "#TODO NOT DONE"
          n19 = call "PhotonPoseEstimator_EstimatePnpDistanceTrigSolvePose.vi"("CameraResult"=w71, "PhotoPoseEstimator"=w72) -> ("Pos Found"=w68:bool, "PhotonEstimatedRobotPose"=w70:T11)  [unwired: 8 in]
          n20 = Not(x=w68) -> (.not. x?=w69:bool)
        }
        frame "CONSTRAINED_SOLVEPNP" {
          # "#TODO NOT DONE"
          n21 = call "PhotonPoseEstimator_Strategy_constrainedPnpStrategy.vi"("CameraResult"=w76, "PhotoPoseEstimator"=w77) -> ("Pos Found"=w73:bool, "PhotonEstimatedRobotPose"=w75:T11)  [unwired: 8 in]
          n22 = Not(x=w73) -> (.not. x?=w74:bool)
        }
      }
    }
  }
  n23 = case shown="True" w13 {
    tunnel: [w80 w81] -> w11
    tunnel: w12 -> [w80 _]
    tunnel: w10 -> [w79 _]
    tunnel: [w79 w82] -> w9
    tunnel: w8 -> [w78 w86]
    tunnel: [w78 w83] -> w7
    tunnel: "PipelineResult" -> [_ w85]
    tunnel: w6 -> [_ w84]
    frame False {
    }
    frame True {
      n24 = case shown="\"CLOSEST_TO_LAST_POSE\"" w84 {
        tunnel: w85 -> [w87 w91 w95 w101 w106 w112 w114 w118 w122]
        tunnel: w86 -> [w88 w92 w96 w105 w107 w113 w115 w119 w123]
        tunnel: [w88 w92 w96 w100 w107 w113 w115 w119 w123] -> w83
        tunnel: [w90 w93 w97 w102 w108 w110 w116 w120 w124] -> w81
        tunnel: [w89 w94 w98 w103 w109 w111 w117 w121 w125] -> w82
        frame "LOWEST_AMBIGUITY" {
          n25 = call "PhotonPoseEstimator_EstimateLowestAmbiguityPose.vi"("CameraResult"=w87, "PhotoPoseEstimator"=w88) -> ("Pos Found"=w90:bool, "PhotonEstimatedRobotPose"=w89:T11)  [unwired: 8 in]
        }
        frame "CLOSEST_TO_CAMERA_HEIGHT" {
          n26 = call "PhotonPoseEstimator_EstimateClosestToCameraHeightPose.vi"("CameraResult"=w91, "PhotoPoseEstimator"=w92) -> ("Pos Found"=w93:bool, "PhotonEstimatedRobotPose"=w94:T11)  [unwired: 8 in]
        }
        frame "CLOSEST_TO_REFERENCE_POSE" {
          n27 = call "PhotonPoseEstimator_GetReferencePose.vi"("PhotonPoseEstimator"=w96) -> ("ReferencePose"=w99:T12)  [unwired: 10 in]
          n28 = call "PhotonPoseEstimator_EstimateClosestToReferencePose.vi"("ReferencePose"=w99, "CameraResult"=w95, "PhotoPoseEstimator"=w96) -> ("Pos Found"=w97:bool, "PhotonEstimatedRobotPose"=w98:T11)  [unwired: 7 in]
        }
        frame "CLOSEST_TO_LAST_POSE" {
          n29 = call "PhotonPoseEstimator_GetLastPose.vi"("PhotonPoseEstimator"=w105) -> ("LastPose"=w104:T12)  [unwired: 10 in]
          n30 = call "PhotonPoseEstimator_SetReferencePose.vi"("ReferencePose"=w104, "PhotonPoseEstimator"=w105) -> ("out PhotonPoseEstimator"=w100:T14)  [unwired: 9 in]
          n31 = call "PhotonPoseEstimator_EstimateClosestToLastPose.vi"("LastPose"=w104, "CameraResult"=w101, "PhotoPoseEstimator"=w100) -> ("Pos Found"=w102:bool, "PhotonEstimatedRobotPose"=w103:T11)  [unwired: 7 in]
        }
        frame "AVERAGE_BEST_TARGETS" {
          n32 = call "PhotonPoseEstimator_EstimateAverageBestTargetsPose.vi"("CameraResult"=w106, "PhotoPoseEstimator"=w107) -> ("Pos Found"=w108:bool, "PhotonEstimatedRobotPose"=w109:T11)  [unwired: 8 in]
        }
        frame "MULTI_TAG_PNP_ON_COPROCESSOR" {
          n33 = call "PhotonPoseEstimator_EstimateMultiTagOnCoprocPose.vi"("CameraResult"=w112, "PhotoPoseEstimator"=w113) -> ("Pos Found"=w110:bool, "PhotonEstimatedRobotPose"=w111:T11)  [unwired: 7 in, 1 out]
        }
        frame "MULTI_TAG_PNP_ON_RIO" {
          # "#TODO NOT DONE"
          n34 = call "PhotonPoseEstimator_EstimateMultiTagOnCoprocPose.vi"("CameraResult"=w114, "PhotoPoseEstimator"=w115) -> ("Pos Found"=w116:bool, "PhotonEstimatedRobotPose"=w117:T11)  [unwired: 7 in, 1 out]
        }
        frame "PNP_DISTANCE_TRIG_SOLVE" {
          # "#TODO NOT DONE"
          n35 = call "PhotonPoseEstimator_EstimatePnpDistanceTrigSolvePose.vi"("CameraResult"=w118, "PhotoPoseEstimator"=w119) -> ("Pos Found"=w120:bool, "PhotonEstimatedRobotPose"=w121:T11)  [unwired: 8 in]
        }
        frame "CONSTRAINED_SOLVEPNP" {
          # "#TODO NOT DONE"
          n36 = call "PhotonPoseEstimator_Strategy_constrainedPnpStrategy.vi"("CameraResult"=w122, "PhotoPoseEstimator"=w123) -> ("Pos Found"=w124:bool, "PhotonEstimatedRobotPose"=w125:T11)  [unwired: 8 in]
        }
      }
    }
  }
  "PhotonEstimatedRobotPose" <- w9
  "Pos Found" <- w11
  n37 = case shown="True" w11 {
    tunnel: w7 -> [w127 w132]
    tunnel: [w128 w131] -> w14
    tunnel: w9 -> [_ w130]
    frame False {
      n38 = call "PhotonPoseEstimator_GetEmptyPose.vi"() -> ("EmptyPose"=w126:T12)  [unwired: 11 in]
      n39 = call "PhotonPoseEstimator_SetLastPose.vi"("LastPose"=w126, "PhotonPoseEstimator"=w127) -> ("out PhotonPoseEstimator"=w128:T14)  [unwired: 9 in]
    }
    frame True {
      # "#TODO This appears to have been\nleft out of the JAVA code.."
      n40 = Unbundle By Name(w130) -> ("EstimatedPose"=w129:T12)
      n41 = call "PhotonPoseEstimator_SetLastPose.vi"("LastPose"=w129, "PhotonPoseEstimator"=w132) -> ("out PhotonPoseEstimator"=w131:T14)  [unwired: 9 in]
    }
  }
  "out PhotonPoseEstimator" <- w14
